vi "Parse Configurable Sequence.vi"(8 "error in":errorcluster, 11 "JSON string":string) -> (0 "error out":errorcluster, 3 "Configurable Sequence":T1)   [LabVIEW 2026]
doc: "Parses a configurable sequence JSON document (docs/CONFIGURABLE_STEP_FORMAT.md). Missing keys keep their defaults, which means not configured. Empty steps give error 5001. AF-free."
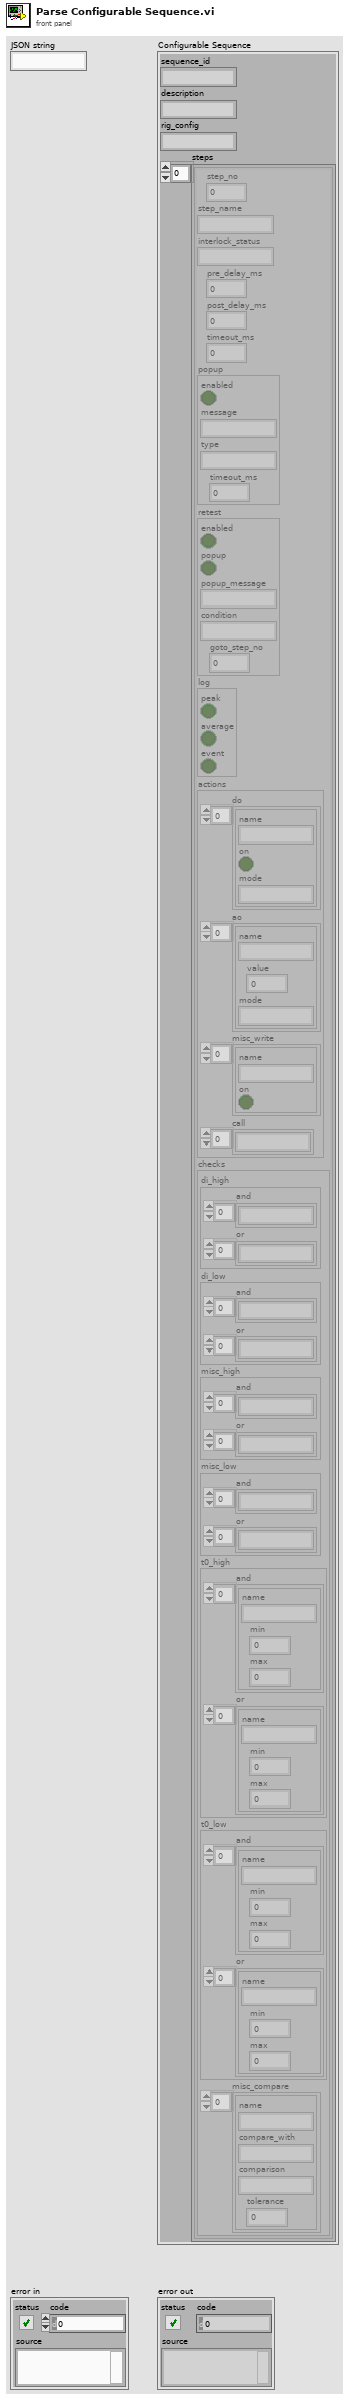
[diagram p1: front panel]
types:
  T1 = cluster{"sequence_id":string, "description":string, "rig_config":string, "steps":cluster{"step_no":i32, "step_name":string, "interlock_status":string, "pre_delay_ms":dbl, "post_delay_ms":dbl, "timeout_ms":dbl, "popup":cluster{"enabled":bool, "message":string, "type":string, "timeout_ms":dbl}, "retest":cluster{"enabled":bool, "popup":bool, "popup_message":string, "condition":string, "goto_step_no":i32}, "log":cluster{"peak":bool, "average":bool, "event":bool}, "actions":cluster{"do":cluster{"name":string, "on":bool, "mode":string}[], "ao":cluster{"name":string, "value":dbl, "mode":string}[], "misc_write":cluster{"name":string, "on":bool}[], "call":string[]}, "checks":cluster{"di_high":cluster{"and":string[], "or":string[]}, "di_low":cluster{"and":string[], "or":string[]}, "misc_high":cluster{"and":string[], "or":string[]}, "misc_low":cluster{"and":string[], "or":string[]}, "t0_high":cluster{"and":cluster{"name":string, "min":dbl, "max":dbl}[], "or":cluster{"name":string, "min":dbl, "max":dbl}[]}, "t0_low":cluster{"and":cluster{"name":string, "min":dbl, "max":dbl}[], "or":cluster{"name":string, "min":dbl, "max":dbl}[]}, "misc_compare":cluster{"name":string, "compare_with":string, "comparison":string, "tolerance":dbl}[]}}[]}
  T2 = cluster{"step_no":i32, "step_name":string, "interlock_status":string, "pre_delay_ms":dbl, "post_delay_ms":dbl, "timeout_ms":dbl, "popup":cluster{"enabled":bool, "message":string, "type":string, "timeout_ms":dbl}, "retest":cluster{"enabled":bool, "popup":bool, "popup_message":string, "condition":string, "goto_step_no":i32}, "log":cluster{"peak":bool, "average":bool, "event":bool}, "actions":cluster{"do":cluster{"name":string, "on":bool, "mode":string}[], "ao":cluster{"name":string, "value":dbl, "mode":string}[], "misc_write":cluster{"name":string, "on":bool}[], "call":string[]}, "checks":cluster{"di_high":cluster{"and":string[], "or":string[]}, "di_low":cluster{"and":string[], "or":string[]}, "misc_high":cluster{"and":string[], "or":string[]}, "misc_low":cluster{"and":string[], "or":string[]}, "t0_high":cluster{"and":cluster{"name":string, "min":dbl, "max":dbl}[], "or":cluster{"name":string, "min":dbl, "max":dbl}[]}, "t0_low":cluster{"and":cluster{"name":string, "min":dbl, "max":dbl}[], "or":cluster{"name":string, "min":dbl, "max":dbl}[]}, "misc_compare":cluster{"name":string, "compare_with":string, "comparison":string, "tolerance":dbl}[]}}[]
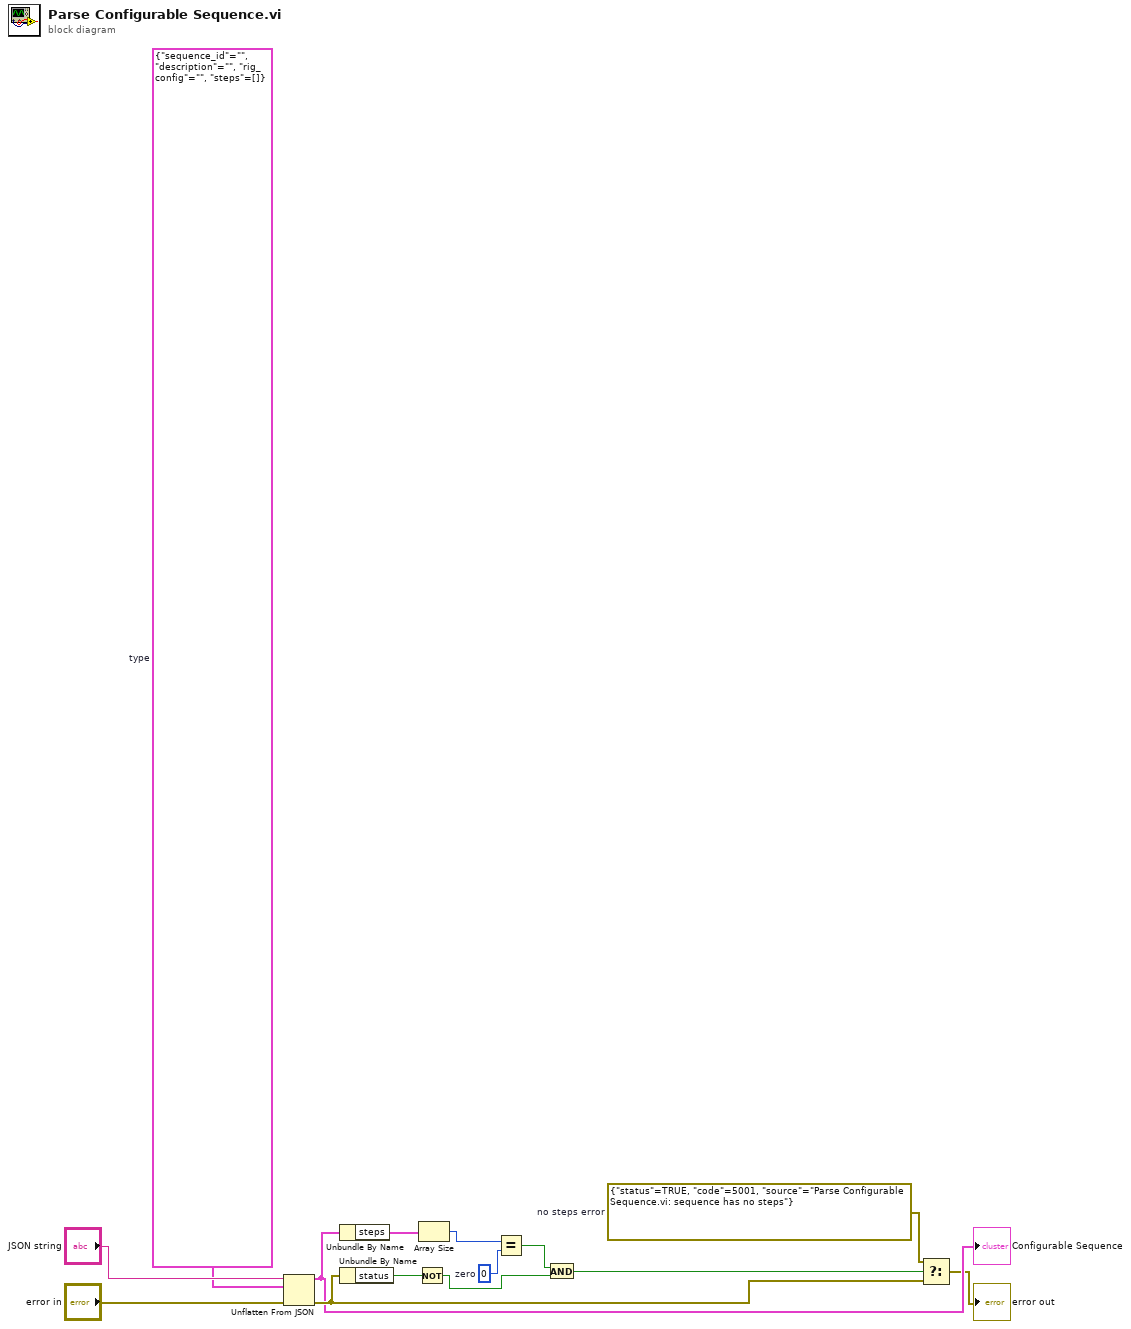
[diagram p0: block diagram]
diagram:
  w5 = errorcluster {"status"=TRUE, "code"=5001, "source"="Parse Configurable Sequence.vi: sequence has no steps"}  # no steps error
  w8 = 0  # zero
  w13 = T1 {"sequence_id"="", "description"="", "rig_config"="", "steps"=[]}  # type
  n1 = Unflatten From JSON(JSON string="JSON string", type and defaults=w13, error in (no error)="error in") -> (value=w2:T1, error out=w3:errorcluster)  [unwired: 4 in]
  "Configurable Sequence" <- w2
  n2 = Unbundle By Name(w2) -> ("steps"=w11:T2)
  n3 = Unbundle By Name(w3) -> ("status"=w10:bool)
  n4 = Not(x=w10) -> (.not. x?=w6:bool)
  n5 = Array Size(array=w11) -> (size(s)=w9:i32)
  n6 = Equal?(x=w9, y=w8) -> (x = y?=w7:bool)
  n7 = And(x=w7, y=w6) -> (x .and. y?=w4:bool)
  n8 = Select(t=w5, s=w4, f=w3) -> (s? t:f=→"error out":errorcluster)
